vi "audio_input.vi"() -> ()   [LabVIEW 2018]
panel:
  out "Data 2":dbl
  out "Data":dynamicdata(graph)
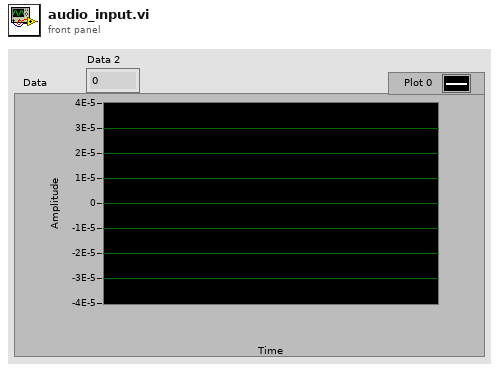
[diagram p1: front panel]
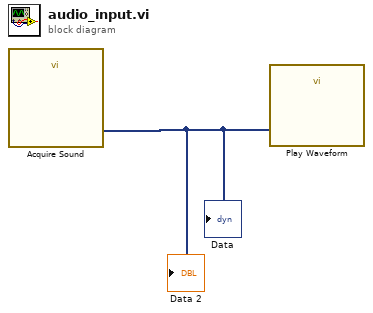
[diagram p0: block diagram]
diagram:
  n1 = call "Acquire Sound"() -> ("Data"=w1:dynamicdata)  [unwired: 18 in, 1 out]
  "Data" <- w1
  "Data 2" <- w1
  n2 = call "Play Waveform"("Data"=w1) -> ()  [unwired: 18 in, 1 out]
